vi "08-send-and-receive-img.vi"() -> ()   [LabVIEW 2018, in "LV2Julia_examples.lvlib"]
uses:
  LV2Julia_examples.lvlib
  LV2Julia_core/VIs/Server or client state.ctl
  LV2Julia_core/VIs/Commands.ctl
  f9264f0d-2c2d-4a22-a0da-9e005a3dfb77.vi
  f9264f0d-2c2d-4a22-a0da-9e005a3dfb77.vi/89b97d22-959e-4b83-8c6b-3c7c62200d75.vi
  f9264f0d-2c2d-4a22-a0da-9e005a3dfb77.vi/89b97d22-959e-4b83-8c6b-3c7c62200d75.vi/744a2648-b7a0-4013-a32a-ced80c55a843.vi
  f9264f0d-2c2d-4a22-a0da-9e005a3dfb77.vi/89b97d22-959e-4b83-8c6b-3c7c62200d75.vi/b7effc4f-98a3-43ca-baee-833fe9a7fa6d.vi
  f9264f0d-2c2d-4a22-a0da-9e005a3dfb77.vi/89b97d22-959e-4b83-8c6b-3c7c62200d75.vi/4accf15f-36e1-4f55-ac4b-8ce4baaa0ee7.vi
  LV2Julia_core/VIs/jl-scripts path.vi
  <vilib>/Utility/error.llb/Error Cluster From Error Code.vi
  LV2Julia_core/VIs/check ID validity.vi
  LV2Julia_core/VIs/bindata_descr to JSON.vi
  LV2Julia_core/VIs/check cluster field names.vi
  LV2Julia_core/VIs/concat JSON.vi
  LV2Julia_core/VIs/build request.vi
  LV2Julia_core/VIs/Parse server response.vi
  LV2Julia_core/VIs/log jl exceptions.vi
  <vilib>/ErrorRing/Error Ring.xnode
  LV2Julia_core/LV2Julia_core.lvlib
panel:
  in  "Transform":T1
  out "picture sent":picture
  in  "image file path":path=path "../other_files/peppers_color_256.png"
  out "picture received":picture
  out "short error info":string
  in  "next":bool
  out "current error":errorcluster
  out "final error":errorcluster
  in  "stop":bool
  out "ZMQ timeout":bool
  out "Julia script file path":path
  out "temporary script path":path
  out "Jl Server state":T2
  # "If you don't see any received picture. check the scrollbars!"
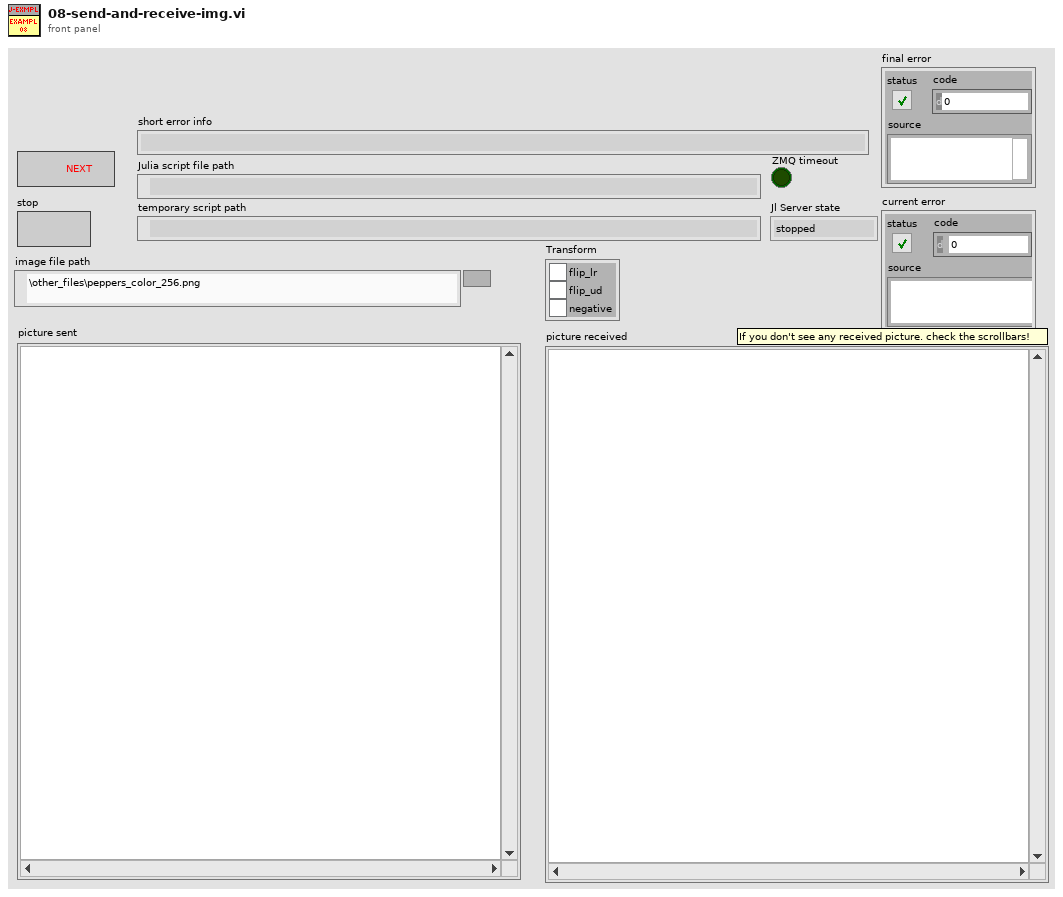
[diagram p1: front panel]
types:
  T1 = cluster{"flip_lr":bool, "flip_ud":bool, "negative":bool}
  T2 = typedef "LV2Julia_core.lvlib/Server or client state.ctl" = enum16{"stopped", "running", "unknown"}
  T3 = typedef "LV2Julia_core.lvlib/Commands.ctl" = enum16{"Start Jl-server & Init LV-client", "Send request & Get response ", "Stop Jl-server & Cleanup LV-client", "Cleanup LV-client", "Start Jl-server", "Stop Jl-server", "Init LV-Client", "Cleanup LV-Client", "(not allowed)", "Set LV Client state", "Set Jl Server state", "set ZMQ timeout", "read ZMQ timeout", "read-out state"}
  T4 = typedef "LV2Julia_core.lvlib/detailed error info.ctl" = cluster{"exception_or_info":string, "trace":T5[]}
  T5 = typedef "LV2Julia_core.lvlib/StackFrame.ctl" = cluster{"frame_summary":string, "func":string, "linfo":string, "file":string, "line":i32, "pointer":u64, "from_c":bool, "inlined":bool}
  T6 = typedef "imagedata.ctl" = cluster{"image type":i32, "image depth":i32, "image":u8[], "mask":u8[], "colors":u32[], "Rectangle":cluster{"left":i16, "top":i16, "right":i16, "bottom":i16}}
  T7 = typedef "LV2Julia_core.lvlib/Bindata&description.ctl" = cluster{"bindata_descr":T8[], "bindata":u8[]}
  T8 = typedef "LV2Julia_core.lvlib/Bindata description.ctl" = cluster{"nofbytes":i32, "numtype":string, "start":i32, "arrdims":i32[], "kwarg_name":string, "category":string}
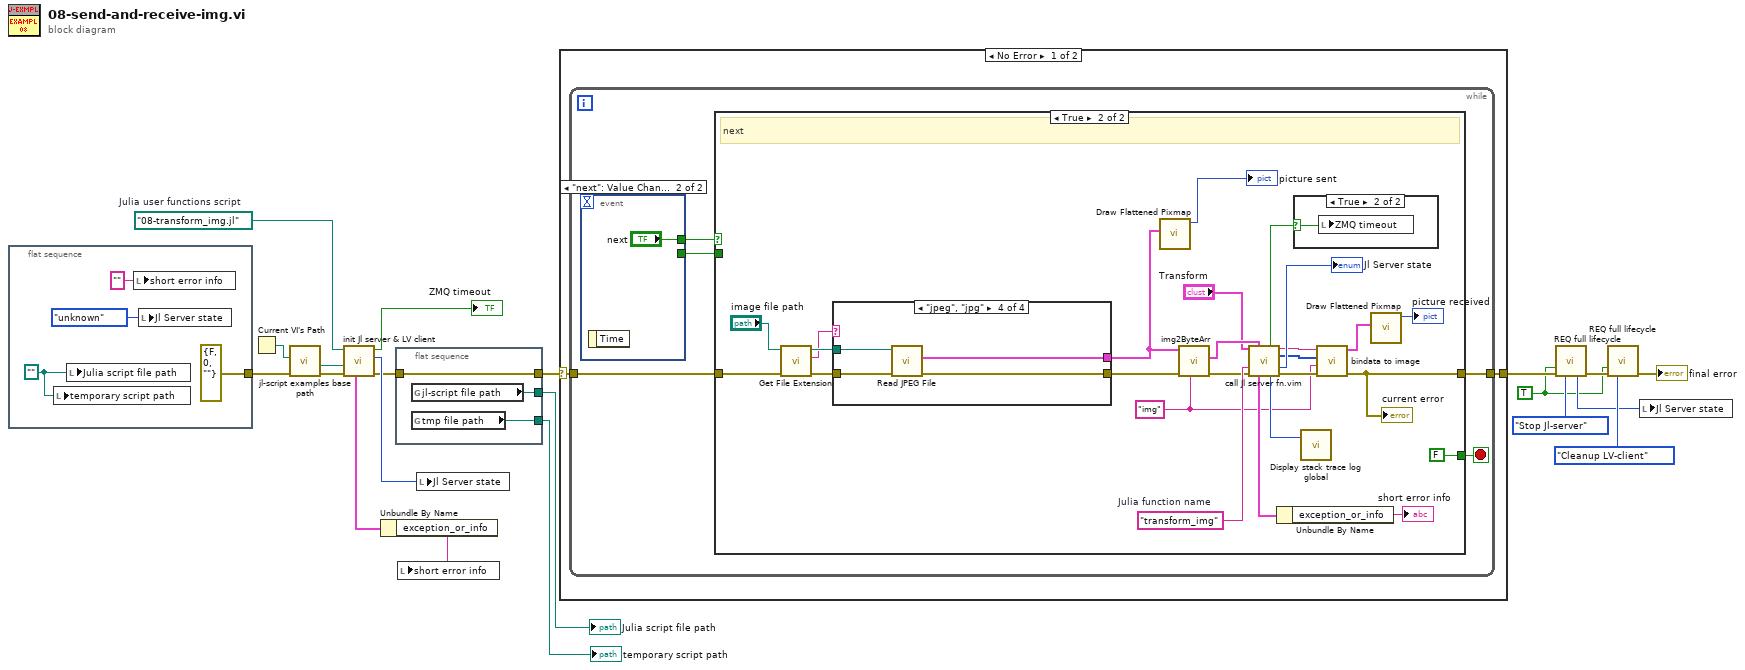
[diagram p0: block diagram]
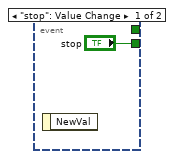
[diagram p2: hidden frame]
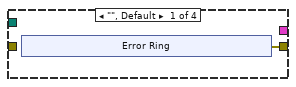
[diagram p4: hidden frame]
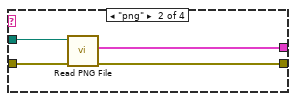
[diagram p5: hidden frame]
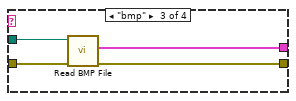
[diagram p6: hidden frame]
diagram:
  w8 = path "08-transform_img.jl"  # Julia user functions script
  w11 = TRUE ("Force command")
  n1 = flat-sequence {
    tunnel: [errorcluster {"status"=FALSE, "code"=0, "source"=""} ("error in (no error)")] -> w4
    frame #0 {
      w22 = path ""
      n2 = local write "temporary script path"(w22) -> ()
      n3 = local write "Julia script file path"(w22) -> ()
      n4 = local write "short error info"("" ("short error info")) -> ()
      n5 = local write "Jl Server state"(Server_or_client_state."unknown" ("Jl Server state out")) -> ()
    }
  }
  n6 = Current VI's Path() -> (path=w6:path)
  n7 = call "jl-script examples base path.vi"("error in (no error)"=w4, "calling example VI path"=w6) -> ("error out"=w5:errorcluster, "jl-script-examples base path"=w3:path)  [unwired: 8 in]
  n8 = call "init Jl server & LV client.vi"("error in (no error)"=w5, "Base path (not a path)"=w3, "Julia user functions script"=w8) -> ("error out"=w7:errorcluster, "Jl Server state out"=w9:T2, "timeout?"=→"ZMQ timeout":bool, "detailed error info"=w1:T4)  [unwired: 3 in, 2 out]
  n9 = Unbundle By Name(w1) -> ("exception_or_info"=w2:string)
  n10 = flat-sequence {
    tunnel: [w27] -> w15
    tunnel: w7 -> [w27]
    tunnel: [w26] -> w13
    tunnel: [w25] -> w14
    frame #0 {
      n11 = global read "jl-scripts path.vi" "jl-script file path"() -> (w26:path)
      n12 = global read "jl-scripts path.vi" "tmp file path"() -> (w25:path)
    }
  }
  n13 = local write "short error info"(w2) -> ()
  n14 = local write "Jl Server state"(w9) -> ()
  n15 = case shown="No Error" w15 {
    selector: w15 -> [w28 w83]
    tunnel: [w29 w83] -> w20
    frame No Error {
      n16 = while {
        tunnel: w28 -> [w33]
        tunnel: [w34] -> w29
        stop <- w31 stop-if-true
        n17 = event shown="[1] \"next\": Value Change" {
          selector: _ -> [_ _]
          dyn-events: _ -> [_ _]
          timeout: _ -> [_ _]
          tunnel: [_ "next"] -> w32
          tunnel: ["stop" _] -> w30
          event "stop": Value Change {
            n18 = event-data() -> ()  [unwired: 1 in, 1 out]
          }
          event "next": Value Change {
            n19 = event-data() -> ()  [unwired: 1 in, 1 out]
          }
        }
        n20 = case shown="True" w32 {
          tunnel: [w38 w53] -> w34
          tunnel: w33 -> [w38 w44]
          tunnel: [w37 FALSE ("stop this VI only")] -> w31
          tunnel: w30 -> [w37 _]
          frame False {
            # "stop"
          }
          frame True {
            w42 = "img" ("name")
            w62 = "transform_img"  # Julia function name
            # "next"
            n21 = call <vilib>:"Get File Extension.vi"("error in (no error)"=w44, "file"="image file path") -> ("error out"=w47:errorcluster, "lowercase file extension"=w45:string, "dup file"=w48:path)  [unwired: 5 in, 2 out]
            n22 = case shown="\"jpeg\", \"jpg\"" w45 {
              tunnel: [_ w73 w77 w81] -> w50
              tunnel: w48 -> [_ w72 w76 w80]
              tunnel: w47 -> [_ w71 w75 w79]
              tunnel: [w64 w70 w74 w78] -> w46
              frame "", Default {
                n23 = xnode "Error Ring"() -> ("error out"=w64:errorcluster)
              }
              frame "png" {
                n24 = call <vilib>:"Read PNG File.vi"("error in (no error)"=w71, "path to PNG file"=w72) -> ("error out"=w70:errorcluster, "image data"=w73:T6)  [unwired: 7 in, 1 out]
              }
              frame "bmp" {
                n25 = call <vilib>:"Read BMP File.vi"("error in (no error)"=w75, "path to BMP file"=w76) -> ("error out"=w74:errorcluster, "image data"=w77:T6)  [unwired: 7 in, 1 out]
              }
              frame "jpeg", "jpg" {
                n26 = call <vilib>:"Read JPEG File.vi"("error in (no error)"=w79, "path to JPEG file"=w80) -> ("error out"=w78:errorcluster, "image data"=w81:T6)  [unwired: 7 in, 1 out]
              }
            }
            n27 = call <vilib>:"Draw Flattened Pixmap.vi"("image data"=w50) -> ("new picture"=→"picture sent":picture)  [unwired: 8 in]
            n28 = call "img2ByteArr.vi"("kwarg_name"=w42, "error in (no error)"=w46, "img in"=w50) -> ("error out"=w43:errorcluster, "Bindata & descr out"=w40:T7)  [unwired: 6 in, 1 out]
            n29 = call "call Jl server fn.vim"("Arguments 1"="Transform", "Bindata & descr in"=w40, "fun2call"=w62, "error in (no error)"=w43) -> ("timeout?"=w60:bool, "JSON received"=w52:string, "binary data received"=w51:u8[], "Jl Server state out"=→"Jl Server state":T2, "detailed error info"=w58:T4, "return code"=w59:u8, "error out"=w54:errorcluster)  [unwired: 5 in]
            n30 = Unbundle By Name(w58) -> ("exception_or_info"=→"short error info":string)
            n31 = case shown="True" w60 {
              selector: w60 -> [_ w82]
              frame False {
              }
              frame True {
                n32 = local write "ZMQ timeout"(w82) -> ()
              }
            }
            n33 = call "Display stack trace log global.vi"("server return code"=w59) -> ()  [unwired: 3 in]
            n34 = call "bindata to image.vi"("error in (no error)"=w54, "name"=w42, "binary data in"=w51, "JSON in"=w52) -> ("error out"=w53:errorcluster, "img out"=w55:T6)  [unwired: 6 in]
            "current error" <- w53
            n35 = call <vilib>:"Draw Flattened Pixmap.vi"("image data"=w55) -> ("new picture"=→"picture received":picture)  [unwired: 8 in]
          }
        }
      }
    }
    frame Error {
    }
  }
  n36 = call "REQ full lifecycle.vi"("Force command"=w11, "error in"=w20, "command"=Commands."Stop Jl-server") -> ("Jl Server state out"=w12:T2, "error out"=w18:errorcluster)  [unwired: 6 in, 5 out]
  n37 = call "REQ full lifecycle.vi"("Force command"=w11, "error in"=w18, "command"=Commands."Cleanup LV-client") -> ("error out"=→"final error":errorcluster)  [unwired: 6 in, 6 out]
  n38 = local write "Jl Server state"(w12) -> ()
  "temporary script path" <- w14
  "Julia script file path" <- w13
